vi "Write CSV File.vi"   [LabVIEW 2013, in "Robust CSV.lvlib"]
uses:
  Robust CSV.lvlib
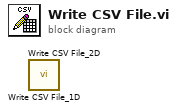
[diagram p0: block diagram]
diagram:
  n1 = call "Write CSV File_1D.vi"() -> ()  [unwired: 10 in, 2 out]
  n2 = call "Write CSV File_2D.vi"() -> ()  [unwired: 10 in, 2 out]
